vi "Stop Core.vi"(10 "final error code":i32, 11 "G-CLI Runner in":refnum<class "Runner.lvclass">) -> (3 "G-CLI Runner out":refnum<class "Runner.lvclass">)   [LabVIEW 2026, in "Runner.lvlib" / "Runner.lvclass"]
doc: "<p>(<strong>Filename</strong>: <span class=\"dnl\">Actor Framework.lvlib:Actor.lvclass:Stop Core.vi</span>)</p>\n<p>Defines what the actor does before it stops. Use the <strong>final error code</strong> input to determine whether the actor shut down in response to an error.</p>\n<p>By default, this method passes the Stop message along to all <a href=\"nihelplauncher://docs/csh?context=lvcore_lvcomm_af_launch_nested_actor\">auto-stop nested actors</a>. A descendant class may override this method to define additional behavior, such as shutting down any processes the actor initiated in its override of the <a href=\"nihelplauncher://docs/csh?context=lvcore_lvcomm_af_actor_core\">Actor Core</a> method.</p>"
uses:
  Runner.lvclass
  Runner.lvclass/Runner.ctl
  <vilib>/ActorFramework/Actor/Actor.lvclass
  <vilib>/ActorFramework/Stop Msg/Stop Msg.lvclass
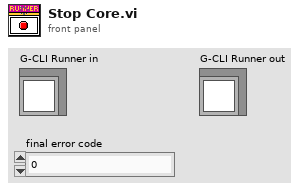
[diagram p1: front panel]
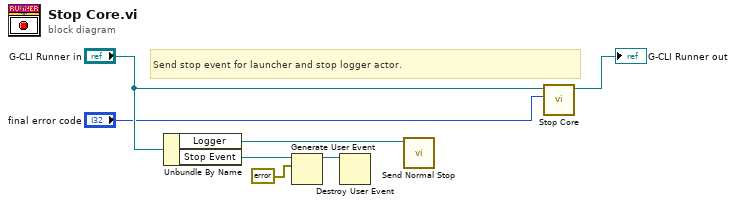
[diagram p0: block diagram]
diagram:
  # "Send stop event for launcher and stop logger actor."
  n1 = Unbundle By Name("G-CLI Runner in") -> ("Logger"=w2:refnum<class "Message Enqueuer.lvclass">, "Stop Event"=w4:refnum<user-event>)
  n2 = Generate User Event(user event=w4, event data cluster=errorcluster {"status"=FALSE, "code"=0, "source"=""} ("error constant")) -> (user event out=w3:refnum<user-event>)  [unwired: 2 in, 1 out]
  n3 = Destroy User Event(user event=w3) -> ()  [unwired: 1 in, 1 out]
  n4 = call <vilib>:"Send Normal Stop.vi"("Message Enqueuer"=w2) -> ()  [unwired: 10 in, 1 out]
  n5 = call-parent "Stop Core.vi"("final error code"="final error code", "Actor in"="G-CLI Runner in") -> ("Actor out"=→"G-CLI Runner out":refnum<class "Runner.lvclass">)  [unwired: 9 in]
